vi "RemoteVI Yield If Idle.vi"(0 "accepted?":bool, 5 "captured?":bool) -> ()   [LabVIEW 2020, in "RemoteVI.lvlib"]
doc: "Waits 1 ms unless the server loop accepted a connection or made a frame in this iteration (busy? TRUE): an idle loop yields the CPU, a busy one goes on at once."
uses:
  RemoteVI.lvlib
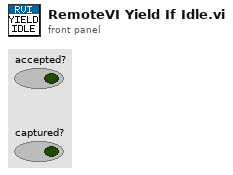
[diagram p1: front panel]
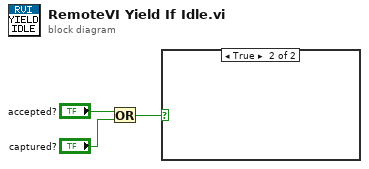
[diagram p0: block diagram]
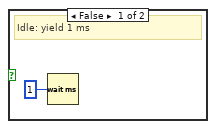
[diagram p2: hidden frame]
diagram:
  n1 = Or(x="accepted?", y="captured?") -> (x .or. y?=w3:bool)
  n2 = case shown="True" w3 {
    frame False {
      # "Idle: yield 1 ms"
      n3 = Wait (ms)(milliseconds to wait=1) -> ()  [unwired: 1 out]
    }
    frame True {
    }
  }
